vi "Wait for Response Message.vi"(6 "Synchronous Request Callback":refnum<class "Synchronous Request Callback.lvclass">, 8 "error in (no error)":errorcluster, 9 "timeout in ms":i32, 11 "Process In":refnum<class "Process.lvclass">) -> (0 "error out":errorcluster, 1 "Message Data":variant, 2 "Message":string, 3 "Process Out":refnum<class "Process.lvclass">, 4 "timed out?":bool)   [LabVIEW 2020, in "Process.lvclass"]
uses:
  Process.lvclass
  Synchronous Request Callback/Synchronous Request Callback.lvclass
  Process.lvclass/Process.ctl
  <vilib>/Utility/error.llb/Error Cluster From Error Code.vi
  <vilib>/ErrorRing/Error Ring.xnode
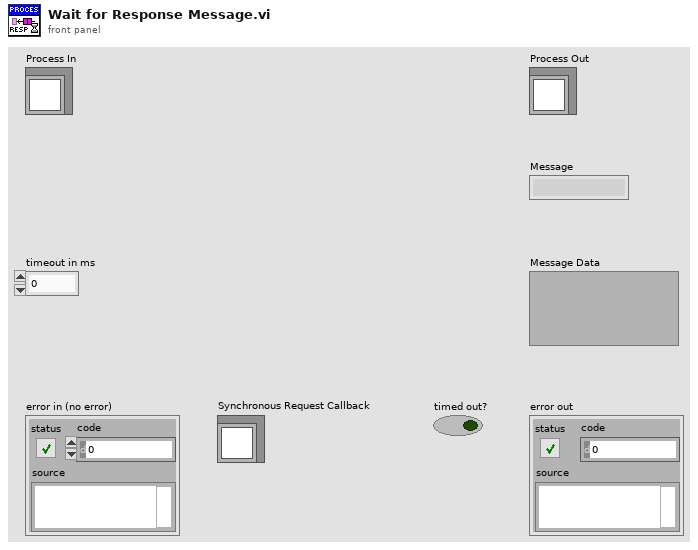
[diagram p1: front panel]
types:
  T1 = typedef "Process.lvclass/Lifecycle State.ctl" = enum16{"Uninitialized", "Initialized", "Started", "Running", "Stopped", "Finished"}
  T2 = typedef "Synchronous Request Callback.lvclass/Response Message Cluster.ctl" = cluster{"Message":string, "Message Data":variant, "Error Out":errorcluster}
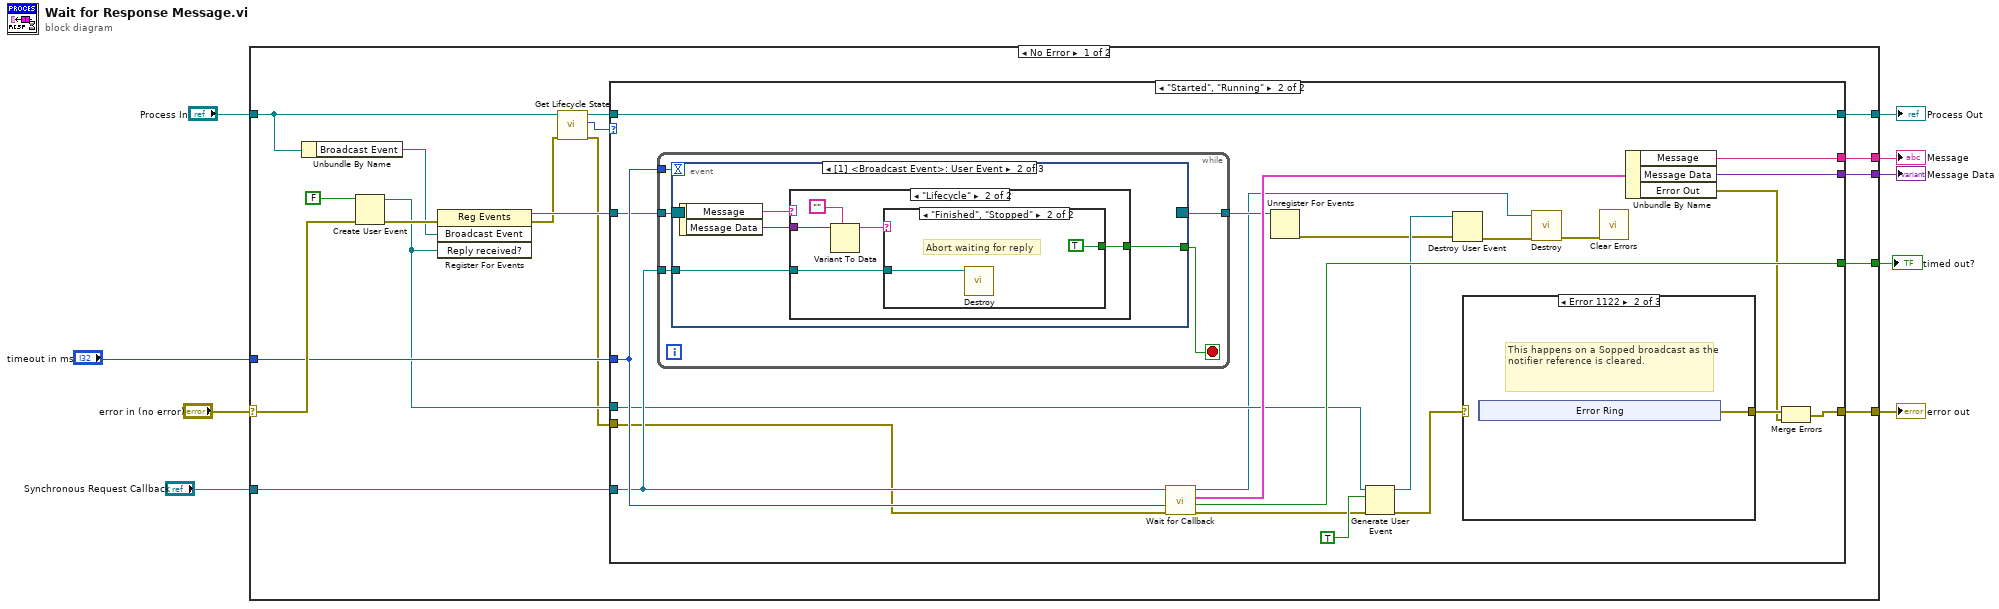
[diagram p0: block diagram]
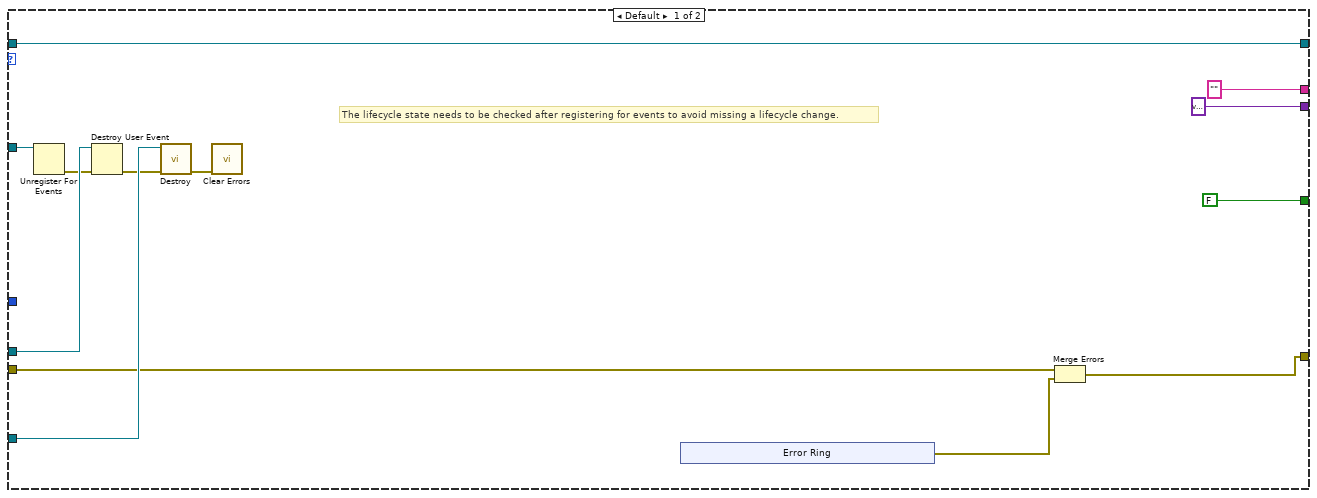
[diagram p2: hidden frame]
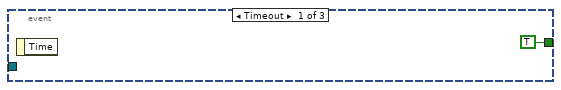
[diagram p5: hidden frame]
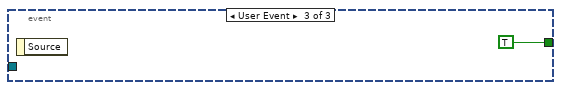
[diagram p8: hidden frame]
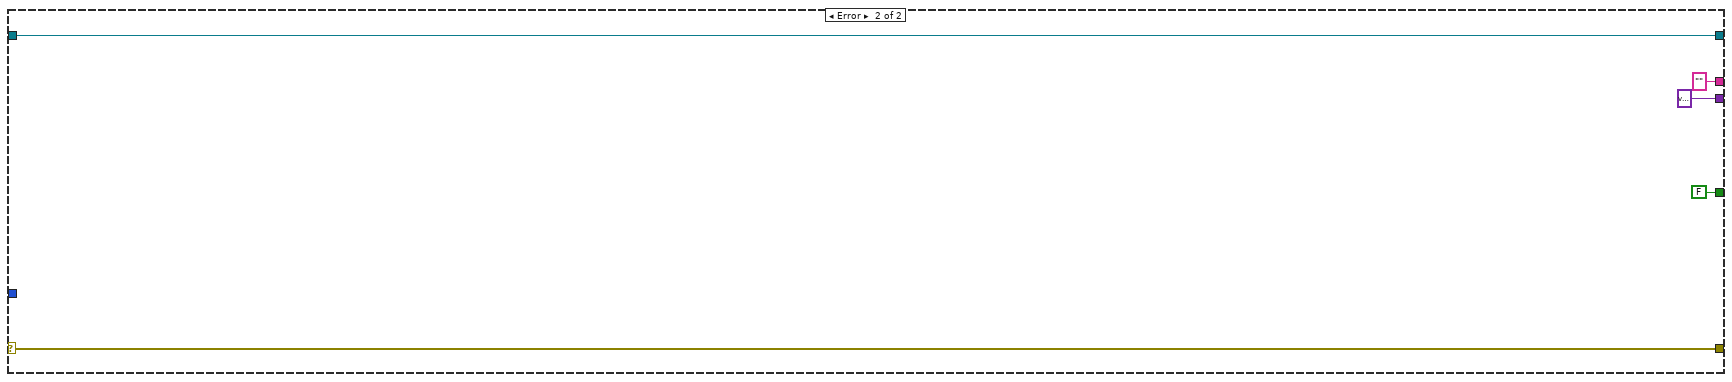
[diagram p9: hidden frame]
diagram:
  n1 = case shown="No Error" "error in (no error)" {
    selector: "error in (no error)" -> [w27 w99]
    tunnel: "timeout in ms" -> [w24 _]
    tunnel: [w22 variant ("Message Data")] -> w7
    tunnel: [w21 "" ("Message")] -> w6
    tunnel: [w20 FALSE ("timed out?")] -> w5
    tunnel: "Process In" -> [w19 w100]
    tunnel: [w18 w99] -> w3
    tunnel: [w13 w100] -> w2
    tunnel: "Synchronous Request Callback" -> [w10 _]
    frame No Error {
      n2 = Unbundle By Name(w19) -> ("Broadcast Event"=w16:refnum<user-event>)
      n3 = Create User Event(user event datatype=FALSE ("Reply received?"), error in=w27) -> (user event=w17:refnum<user-event>, error out=w26:errorcluster)
      n4 = register-events(error in=w26, w16, w17) -> (reference out=w23:refnum<event-registration>, error out=w15:errorcluster)  [unwired: 1 in]
      n5 = call "Get Lifecycle State.vi"("error in (no error)"=w15, "Process In"=w19) -> ("error out"=w14:errorcluster, "Lifecycle State"=w11:T1, "Process Out"=w12:refnum<class "Process.lvclass">)  [unwired: 6 in, 1 out]
      n6 = case shown="\"Started\", \"Running\"" w11 {
        tunnel: w24 -> [_ w66]
        tunnel: w23 -> [w34 w65]
        tunnel: [variant ("Message Data") w64] -> w22
        tunnel: ["" ("Message") w63] -> w21
        tunnel: [FALSE ("timed out?") w61] -> w20
        tunnel: w10 -> [w32 w60]
        tunnel: [w39 w46] -> w18
        tunnel: w17 -> [w33 w56]
        tunnel: w14 -> [w29 w48]
        tunnel: [w40 w47] -> w13
        tunnel: w12 -> [w40 w47]
        frame Default {
          # "The lifecycle state needs to be checked after registering for events to avoid missing a lifecycle change."
          n7 = Unregister For Events(event registration refnum=w34) -> (error out=w31:errorcluster)  [unwired: 1 in]
          n8 = Destroy User Event(user event=w33, error in=w31) -> (error out=w30:errorcluster)
          n9 = call "Destroy.vi"("error in (no error)"=w30, "Synchronous Request Callback In"=w32) -> ("error out"=w28:errorcluster)  [unwired: 9 in]
          n10 = call <vilib>:"Clear Errors.vi"("error in (no error)"=w28) -> ()  [unwired: 5 in, 2 out]
          n11 = xnode "Error Ring"() -> ("error out"=w38:errorcluster)
          n12 = Merge Errors(w29, w38) -> (w39:errorcluster)
        }
        frame "Started", "Running" {
          n13 = while {
            tunnel: w65 -> [w82]
            tunnel: w66 -> [w81]
            tunnel: w60 -> [w79]
            tunnel: [w78] -> w59
            stop <- w80 stop-if-true
            n14 = event shown="[1] <Broadcast Event>: User Event" {
              selector: w82 -> [_ _ _]
              dyn-events: [_ _ _] -> w78
              timeout: w81 -> [_ _ _]
              tunnel: [TRUE w84 TRUE] -> w80
              tunnel: w79 -> [_ w85 _]
              event Timeout {
                n15 = event-data() -> ()  [unwired: 1 in, 1 out]
              }
              event User Event {
                n16 = event-data() -> ("Message"=w87:string, "Message Data"=w86:variant)  [unwired: 1 in]
                n17 = case shown="\"Lifecycle\"" w87 {
                  tunnel: w86 -> [_ w92]
                  tunnel: w85 -> [_ w89]
                  tunnel: [_ w88] -> w84
                  frame Default {
                  }
                  frame "Lifecycle" {
                    n18 = Variant To Data(type="", Variant=w92) -> (data=w90:string)  [unwired: 1 in, 1 out]
                    n19 = case shown="\"Finished\", \"Stopped\"" w90 {
                      tunnel: w89 -> [_ w94]
                      tunnel: [_ TRUE] -> w88
                      frame Default {
                      }
                      frame "Finished", "Stopped" {
                        # "Abort waiting for reply"
                        n20 = call "Destroy.vi"("Synchronous Request Callback In"=w94) -> ()  [unwired: 10 in, 1 out]
                      }
                    }
                  }
                }
              }
              event User Event {
                n21 = event-data() -> ()  [unwired: 1 in, 1 out]
              }
            }
          }
          n22 = call "Wait for Callback.vi"("error in (no error)"=w48, "timeout in ms (-1)"=w66, "Synchronous Request Callback In"=w60) -> ("error out"=w52:errorcluster, "timed out?"=w61:bool, "notification"=w62:T2, "Synchronous Request Callback Out"=w50:refnum<class "Synchronous Request Callback.lvclass">)  [unwired: 5 in]
          n23 = Unregister For Events(event registration refnum=w59) -> (error out=w54:errorcluster)  [unwired: 1 in]
          n24 = Generate User Event(user event=w56, event data cluster=TRUE ("event data"), error in=w52) -> (user event out=w55:refnum<user-event>, error out=w57:errorcluster)  [unwired: 1 in]
          n25 = Destroy User Event(user event=w55, error in=w54) -> (error out=w51:errorcluster)
          n26 = case shown="Error 1122" w57 {
            selector: w57 -> [w67 _ w77]
            tunnel: [w67 w68 w77] -> w58
            frame No Error {
            }
            frame Error {
              # "This happens on a Sopped broadcast as the notifier reference is cleared."
              n27 = xnode "Error Ring"() -> ()  [unwired: 1 out]
              n28 = xnode "Error Ring"() -> ("error out"=w68:errorcluster)
            }
            frame Default {
            }
          }
          n29 = call "Destroy.vi"("error in (no error)"=w51, "Synchronous Request Callback In"=w50) -> ("error out"=w49:errorcluster)  [unwired: 9 in]
          n30 = call <vilib>:"Clear Errors.vi"("error in (no error)"=w49) -> ()  [unwired: 5 in, 2 out]
          n31 = Unbundle By Name(w62) -> ("Message"=w63:string, "Message Data"=w64:variant, "Error Out"=w45:errorcluster)
          n32 = Merge Errors(w58, w45) -> (w46:errorcluster)
        }
      }
    }
    frame Error {
    }
  }
  "Process Out" <- w2
  "error out" <- w3
  "Message Data" <- w7
  "Message" <- w6
  "timed out?" <- w5
